vi "Tester - Array Size.vi"() -> ()   [LabVIEW 2026, in "RSysUtils Array.lvlib"]
uses:
  RSysUtils Array.lvlib
  01681abc-79dc-42ed-a4fc-6c544cf1da53.vi
  ec157c9b-0cd3-468a-a555-1131a0154307.vi
  a86e8fa6-b5a6-41e6-90d3-6ece77e44d58.vi
  f5a3ced2-6bb5-476f-8297-6f75b9b90859.vi
  8f88f1ef-a89e-4532-a9ec-0951da36afe9.vi
  aa23d5c1-4c13-45f0-b6fe-acc27e8a4f4f.vi
  ac8dca4a-e6eb-4a0d-b57a-9deada1a6149.vi
  9d3f68ae-4da3-49f0-a1a1-9f014f00b50a.vi
panel:
  out "Number of Pages 8":i32
  out "Number of Rows 8":i32
  out "Number of Columns 8":i32
  out "Number of Pages 7":i32
  out "Number of Rows 7":i32
  out "Number of Columns 7":i32
  out "Number of Pages 6":i32
  out "Number of Rows 6":i32
  out "Number of Columns 6":i32
  out "Number of Columns 5":i32
  out "Number of Rows 5":i32
  out "Number of Pages 5":i32
  out "Number of Rows 4":i32
  out "Number of Columns 4":i32
  out "Number of Rows 3":i32
  out "Number of Columns 3":i32
  out "Number of Rows 2":i32
  out "Number of Columns 2":i32
  out "Number of Columns 1":i32
  out "Number of Rows 1":i32
  # "Tester\nGet 2D Array Size.vim\nGet 3D Array Size.vim"
  # "Get 2D Array Size"
  # "Get 3D Array Size"
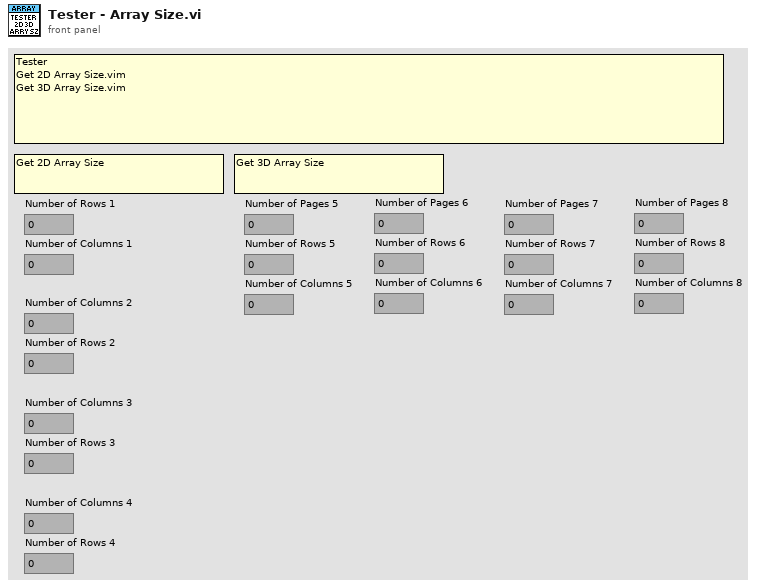
[diagram p1: front panel]
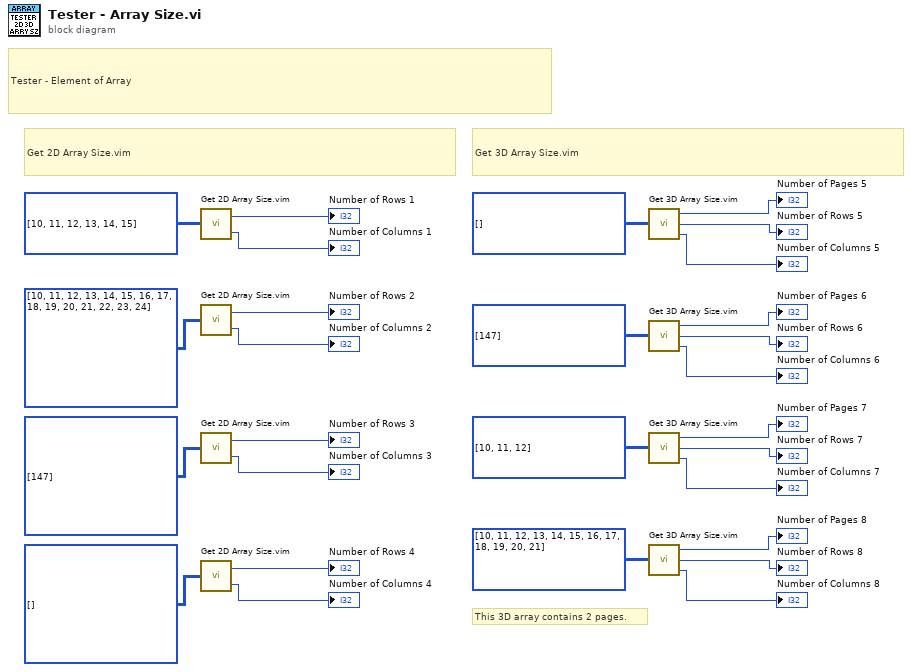
[diagram p0: block diagram]
diagram:
  # "This 3D array contains 2 pages."
  # "Get 3D Array Size.vim"
  # "Get 2D Array Size.vim"
  # "Tester - Element of Array"
  n1 = call "Get 2D Array Size.vim"("2D Array"=i32[][] [[10, 11, 12], [13, 14, 15]]) -> ("Number of Rows"=→"Number of Rows 1":i32, "Number of Columns"=→"Number of Columns 1":i32)
  n2 = call "Get 2D Array Size.vim"("2D Array"=i32[][] [[10, 11, 12], [13, 14, 15], [16, 17, 18], [19, 20, 21], [22, 23, 24]]) -> ("Number of Rows"=→"Number of Rows 2":i32, "Number of Columns"=→"Number of Columns 2":i32)
  n3 = call "Get 2D Array Size.vim"("2D Array"=i32[][] [[147]]) -> ("Number of Rows"=→"Number of Rows 3":i32, "Number of Columns"=→"Number of Columns 3":i32)
  n4 = call "Get 2D Array Size.vim"("2D Array"=i32[][] []) -> ("Number of Rows"=→"Number of Rows 4":i32, "Number of Columns"=→"Number of Columns 4":i32)
  n5 = call "Get 3D Array Size.vim"("3D Array"=i32[][][] []) -> ("Number of Pages"=→"Number of Pages 5":i32, "Number of Rows"=→"Number of Rows 5":i32, "Number of Columns"=→"Number of Columns 5":i32)
  n6 = call "Get 3D Array Size.vim"("3D Array"=i32[][][] [[[147]]]) -> ("Number of Pages"=→"Number of Pages 6":i32, "Number of Rows"=→"Number of Rows 6":i32, "Number of Columns"=→"Number of Columns 6":i32)
  n7 = call "Get 3D Array Size.vim"("3D Array"=i32[][][] [[[10, 11, 12]]]) -> ("Number of Pages"=→"Number of Pages 7":i32, "Number of Rows"=→"Number of Rows 7":i32, "Number of Columns"=→"Number of Columns 7":i32)
  n8 = call "Get 3D Array Size.vim"("3D Array"=i32[][][] [[[10, 11, 12], [13, 14, 15]], [[16, 17, 18], [19, 20, 21]]]) -> ("Number of Pages"=→"Number of Pages 8":i32, "Number of Rows"=→"Number of Rows 8":i32, "Number of Columns"=→"Number of Columns 8":i32)
